vi "Connect TurnTable.vi"(8 "error in (no error)":errorcluster caption="에러 입력(에러 없음)", 10 "VISA resource name":refnum<visa-resource-name>, 11 "Instrument Manager 입력":refnum<class "Instrument Manager.lvclass">) -> (0 "error out":errorcluster caption="에러 출력", 3 "Instrument Manager 출력":refnum<class "Instrument Manager.lvclass">)   [LabVIEW 2023, in "Instrument Manager.lvclass"]
uses:
  Instrument Manager.lvclass
  Module/Turn Table and Mast Control/Class/CO3000/CO3000.lvclass
  C:/Users/HCT-3320/Documents/Instrument Manger/Module/Turn Table and Mast Control/Interface Class/Turn Table/Interface - Turn Table.lvclass
  Instrument Manager.lvclass/Instrument Manager.ctl
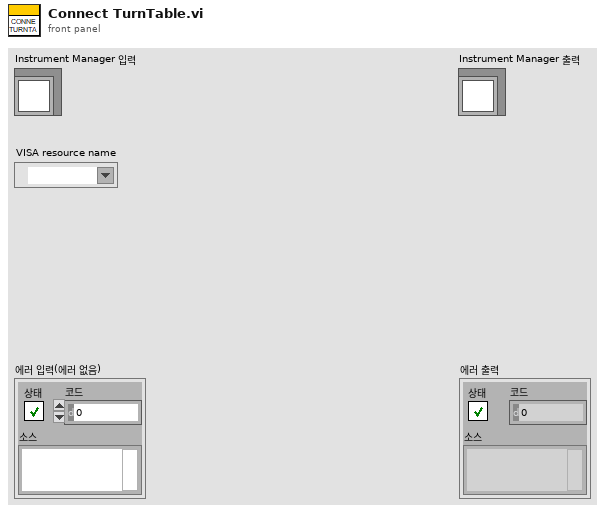
[diagram p1: front panel]
types:
  T1 = cluster{"Anritsu Call Box":refnum<class "Anritsu Call Box.lvclass">, "Spectrum Analyzer":refnum<class "Interface_Spectrum.lvclass">, "RF Switch Box":refnum<class "RF Filter Box.lvclass">, "Turn Table":refnum<class "Interface - Turn Table.lvclass">, "Mast":refnum<class "Interface - Mast.lvclass">, "3D Controller":refnum<class "Interface_3D Controller.lvclass">}
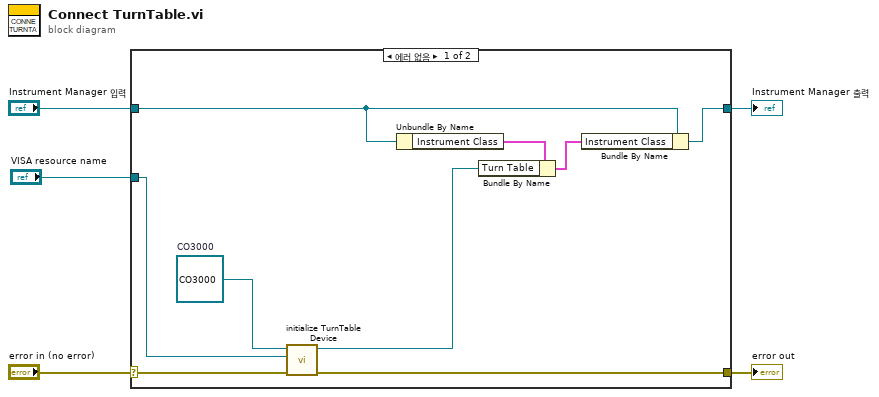
[diagram p0: block diagram]
diagram:
  n1 = case shown="에러 없음" "error in (no error)" {
    selector: "error in (no error)" -> [w7 w16]
    tunnel: [w6 w16] -> w4
    tunnel: [w11 w15] -> w2
    tunnel: "Instrument Manager 입력" -> [w10 w15]
    tunnel: "VISA resource name" -> [w8 _]
    frame No Error {
      w14 = refnum<class "CO3000.lvclass"> refnum  # CO3000
      n2 = call-dynamic "initialize TurnTable Device.vi"("error in (no error)"=w7, "VISA resource name"=w8, "CO3000 in"=w14) -> ("error out"=w6:errorcluster, "CO3000 out"=w9:refnum<class "CO3000.lvclass">)  [unwired: 7 in]
      n3 = Unbundle By Name(w10) -> ("Instrument Class"=w13:T1)
      n4 = Bundle By Name(cluster=w13, "Turn Table"=w9) -> (w12:T1)
      n5 = Bundle By Name(cluster=w10, "Instrument Class"=w12) -> (w11:refnum<class "Instrument Manager.lvclass">)
    }
    frame Error {
    }
  }
  "error out" <- w4
  "Instrument Manager 출력" <- w2
